vi "Enqueue Message Data.vi"(6 "Priority message (F)":bool, 8 "error in (no error)":errorcluster, 9 "Data":variant, 10 "Message":string, 11 "queue in":refnum<queue>) -> (0 "error out":errorcluster, 3 "queue out":refnum<queue>)   [LabVIEW 2021]
uses:
  Type defs/Message cluster.ctl
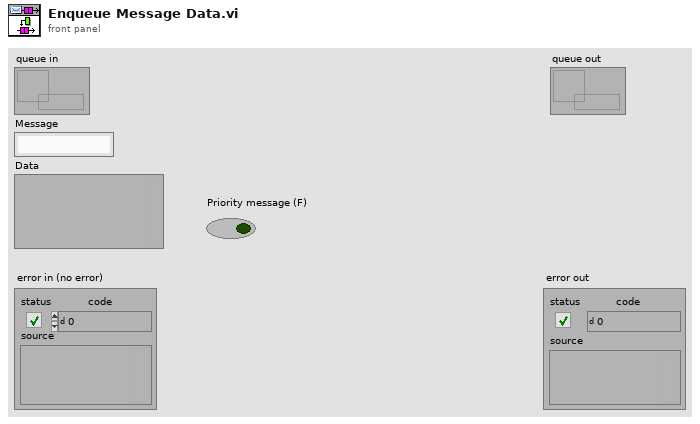
[diagram p1: front panel]
types:
  T1 = typedef "Message cluster.ctl" = cluster{"Message":string, "Data":variant}
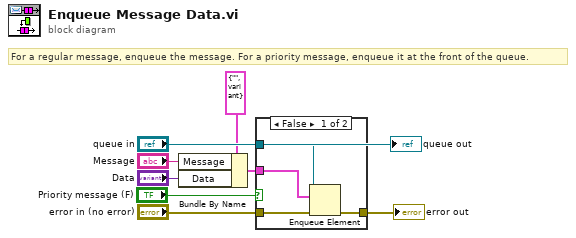
[diagram p0: block diagram]
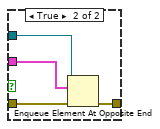
[diagram p2: hidden frame]
diagram:
  # "For a regular message, enqueue the message. For a priority message, enqueue it at the front of the queue."
  n1 = Bundle By Name(cluster=T1 {"Message"="", "Data"=variant} ("Message cluster"), "Message"="Message", "Data"="Data") -> (w6:T1)
  n2 = case shown="False" "Priority message (F)" {
    tunnel: w6 -> [w12 w16]
    tunnel: "queue in" -> [w9 w13]
    tunnel: "error in (no error)" -> [w11 w15]
    tunnel: [w10 w14] -> w3
    frame False {
      n3 = Enqueue Element(queue=w9, element=w12, error in (no error)=w11) -> (error out=w10:errorcluster)  [unwired: 1 in, 2 out]
    }
    frame True {
      n4 = Enqueue Element At Opposite End(queue=w13, element=w16, error in (no error)=w15) -> (error out=w14:errorcluster)  [unwired: 1 in, 2 out]
    }
  }
  "error out" <- w3
  "queue out" <- "queue in"
